vi "Mode selection .vi"(8 "error out":errorcluster) -> (0 "error out 2":errorcluster, 3 "Enum":T1)   [LabVIEW 2021]
uses:
  Control/Mode.ctl
  Control/Set_Get.ctl
panel:
  in  "Back Button":bool
  in  "OFFLINE":bool
  # "SELECT THE MODE"
  # "ONLINE"
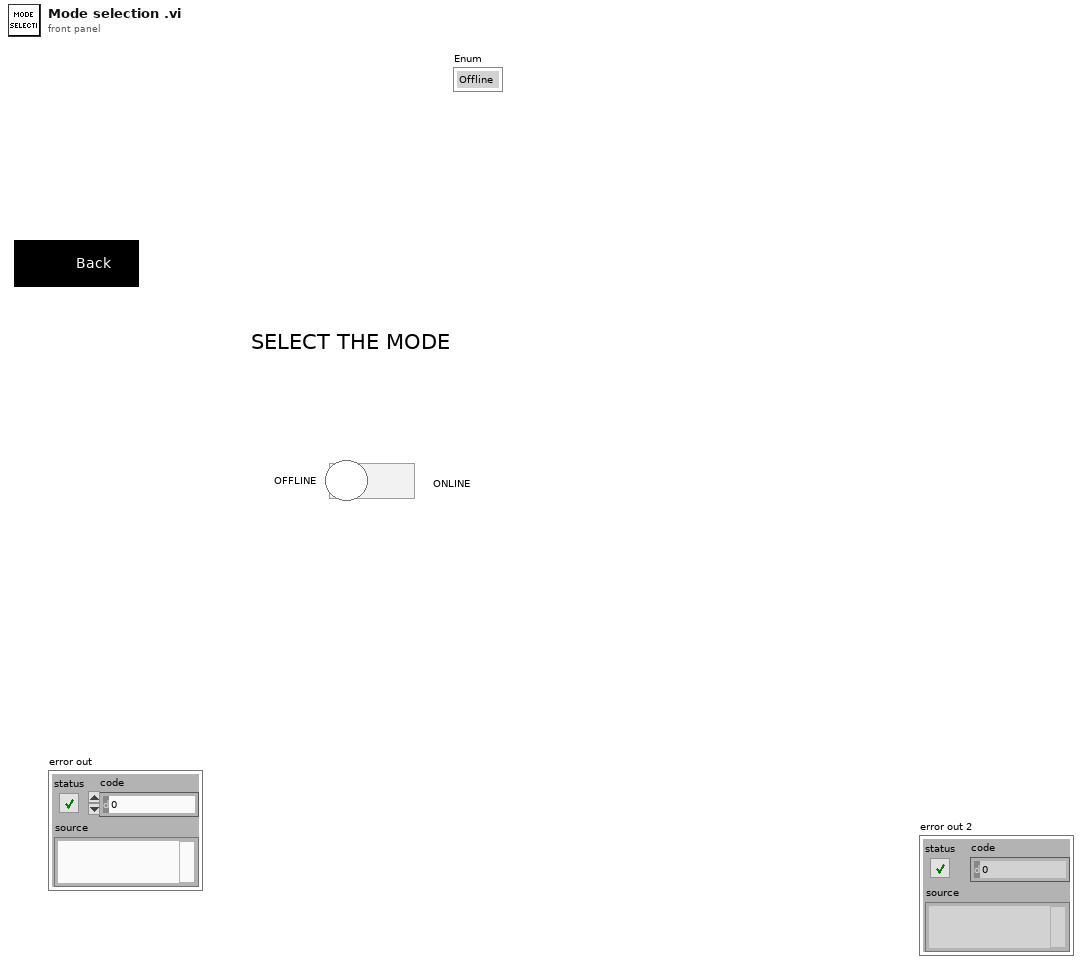
[diagram p1: front panel]
types:
  T1 = typedef "Mode.ctl" = enum16{"Offline", "Online"}
  T2 = typedef "Set_Get.ctl" = enum16{"Set", "Get"}
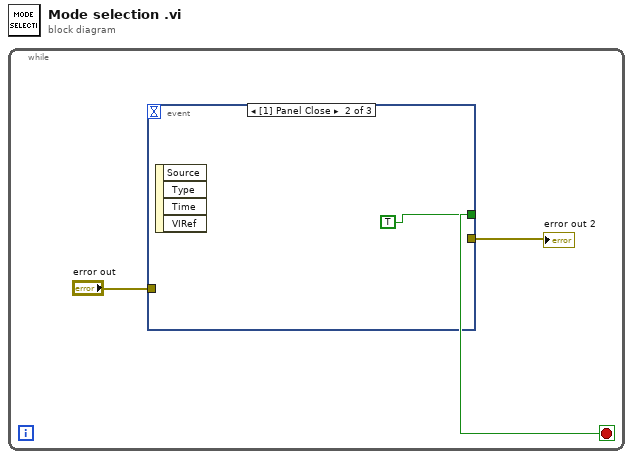
[diagram p0: block diagram]
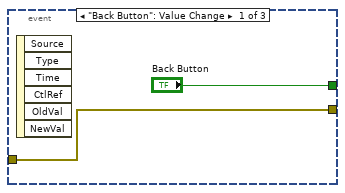
[diagram p2: hidden frame]
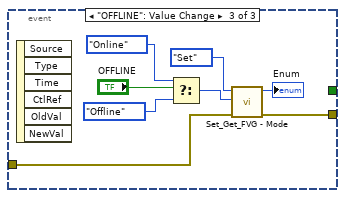
[diagram p3: hidden frame]
diagram:
  n1 = while {
    stop <- w3 stop-if-true
    n2 = event shown="[1] Panel Close" {
      selector: _ -> [_ _ _]
      dyn-events: _ -> [_ _ _]
      timeout: _ -> [_ _ _]
      tunnel: ["Back Button" TRUE _] -> w3
      tunnel: "error out" -> [w4 _ w8]
      tunnel: [w4 _ w7] -> w1
      event "Back Button": Value Change {
        n3 = event-data() -> ()  [unwired: 1 in, 6 out]
      }
      event Panel Close {
        n4 = event-data() -> ()  [unwired: 1 in, 4 out]
      }
      event "OFFLINE": Value Change {
        n5 = event-data() -> ()  [unwired: 1 in, 6 out]
        n6 = Select(t=Mode."Online", s="OFFLINE", f=Mode."Offline") -> (s? t:f=w11:T1)
        n7 = call "Set_Get_FVG - Mode.vi"("error out"=w8, 10:w11, "Enum"=Set_Get."Set") -> ("error out 2"=w7:errorcluster, "Enum"=→"Enum":T1)  [unwired: 7 in]
      }
    }
    "error out 2" <- w1
  }
